vi "String To Number(I32).vi"(5 "String":string) -> (0 "Numeric(I32)":i32)   [LabVIEW 2017]
uses:
  581c0f11-9c78-43f6-8d57-08c5360404ff.vi
  4eae6f33-c0f2-4f9a-9685-dff6b581849e.vi
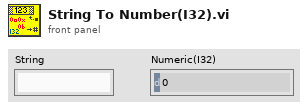
[diagram p1: front panel]
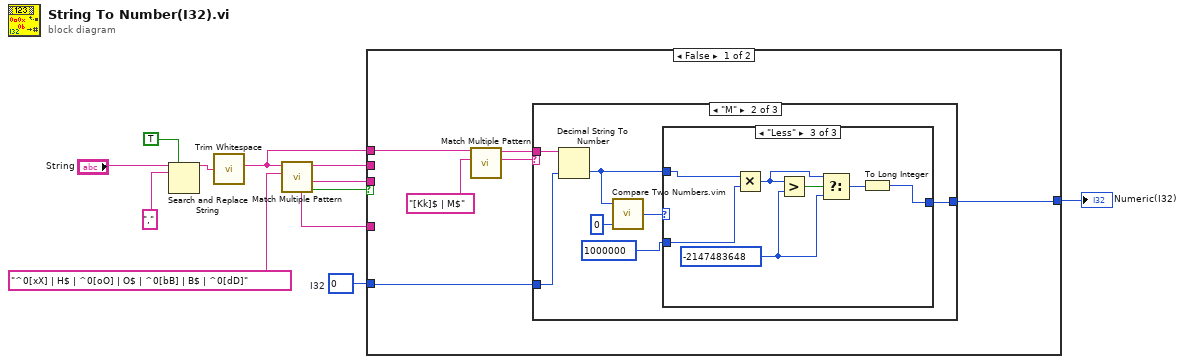
[diagram p0: block diagram]
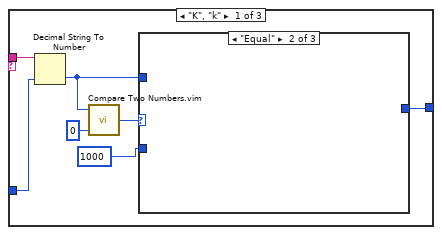
[diagram p2: hidden frame]
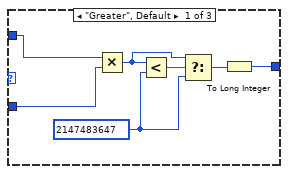
[diagram p3: hidden frame]
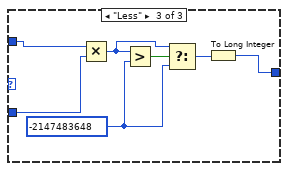
[diagram p4: hidden frame]
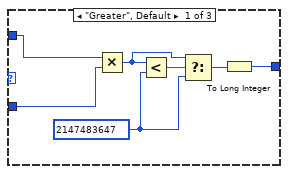
[diagram p5: hidden frame]
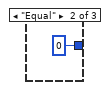
[diagram p6: hidden frame]
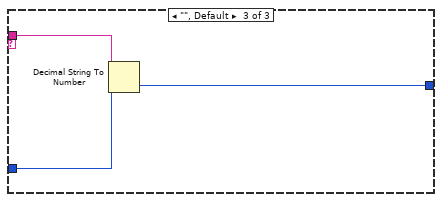
[diagram p7: hidden frame]
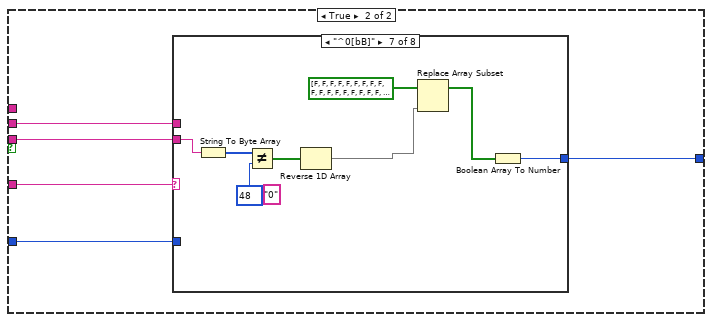
[diagram p8: hidden frame]
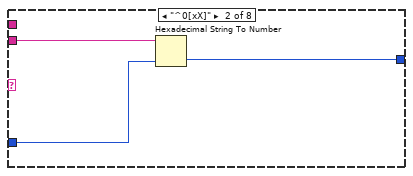
[diagram p10: hidden frame]
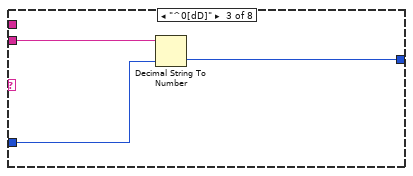
[diagram p11: hidden frame]
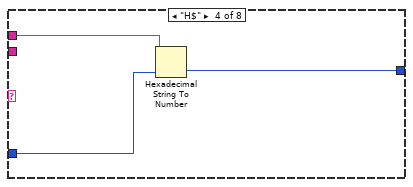
[diagram p12: hidden frame]
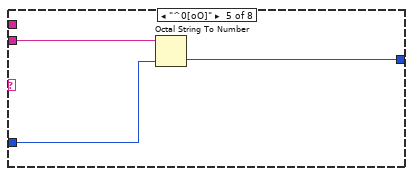
[diagram p13: hidden frame]
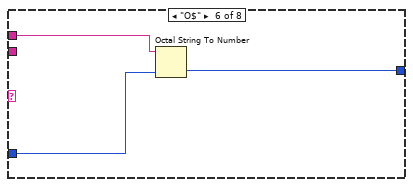
[diagram p14: hidden frame]
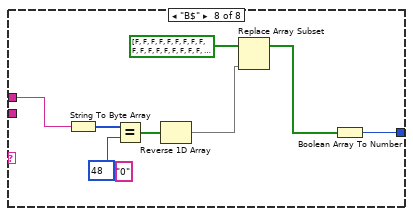
[diagram p15: hidden frame]
diagram:
  w1 = 0  # I32
  n1 = Search and Replace String(replace all?=TRUE ("replace all? (F)"), input string="String", search string=",") -> (result string=w9:string)  [unwired: 5 in, 3 out]
  n2 = call <vilib>:"Trim Whitespace.vi"("string"=w9) -> ("trimmed string"=w2:string)  [unwired: 1 in]
  n3 = call "Match Multiple Pattern.vi"("regular expression"="^0[xX] | H$ | ^0[oO] | O$ | ^0[bB] | B$ | ^0[dD]", "string"=w2) -> ("Found?"=w7:bool, "after substring"=w5:string, "before substring"=w4:string, "pattern matched"=w6:string)  [unwired: 5 in, 1 out]
  n4 = case shown="False" w7 {
    tunnel: w6 -> [_ w69]
    tunnel: w5 -> [_ w68]
    tunnel: w4 -> [_ w67]
    tunnel: [w13 w66] -> w3
    tunnel: w2 -> [w15 _]
    tunnel: w1 -> [w14 w65]
    frame False {
      n5 = call "Match Multiple Pattern.vi"("regular expression"="[Kk]$ | M$", "string"=w15) -> ("match substring"=w17:string, "before substring"=w16:string)  [unwired: 5 in, 3 out]
      n6 = case shown="\"M\"" w17 {
        tunnel: [w22 w43 w64] -> w13
        tunnel: w14 -> [w21 w42 w63]
        tunnel: w16 -> [w25 w46 w62]
        frame "K", "k" {
          n7 = Decimal String To Number(string=w25, default (0L)=w21) -> (number=w20:i32)  [unwired: 1 in, 1 out]
          n8 = call "Compare Two Numbers.vim"("Ref"=0, "Number"=w20) -> ("Result"=w23:enum16{"Greater", "Equal", "Less"})  [unwired: 1 in, 2 out]
          n9 = case shown="\"Equal\"" w23 {
            tunnel: [w26 _ w34] -> w22
            tunnel: w20 -> [w29 _ w35]
            tunnel: u64 1000 ("y") -> [w28 _ w33]
            frame "Greater", Default {
              w30 = 2147483647 ("y")
              n10 = Multiply(x=w29, y=w28) -> (x*y=w31:u64)
              n11 = Less?(x=w31, y=w30) -> (x < y?=w32:bool)
              n12 = Select(t=w31, s=w32, f=w30) -> (s? t:f=w27:u64)
              n13 = To Long Integer(number=w27) -> (32bit integer=w26:i32)
            }
            frame "Equal" {
            }
            frame "Less" {
              w37 = -2147483648 ("y")
              n14 = Multiply(x=w35, y=w33) -> (x*y=w38:u64)
              n15 = Greater?(x=w38, y=w37) -> (0:w39:bool)
              n16 = Select(t=w38, s=w39, f=w37) -> (s? t:f=w36:u64)
              n17 = To Long Integer(number=w36) -> (32bit integer=w34:i32)
            }
          }
        }
        frame "M" {
          n18 = Decimal String To Number(string=w46, default (0L)=w42) -> (number=w41:i32)  [unwired: 1 in, 1 out]
          n19 = call "Compare Two Numbers.vim"("Ref"=0, "Number"=w41) -> ("Result"=w44:enum16{"Greater", "Equal", "Less"})  [unwired: 1 in, 2 out]
          n20 = case shown="\"Less\"" w44 {
            tunnel: [w48 0 w56] -> w43
            tunnel: w41 -> [w50 _ w57]
            tunnel: i64 1000000 ("y") -> [w47 _ w55]
            frame "Greater", Default {
              w51 = 2147483647 ("y")
              n21 = Multiply(x=w50, y=w47) -> (x*y=w52:i64)
              n22 = Less?(x=w52, y=w51) -> (x < y?=w53:bool)
              n23 = Select(t=w52, s=w53, f=w51) -> (s? t:f=w49:i64)
              n24 = To Long Integer(number=w49) -> (32bit integer=w48:i32)
            }
            frame "Equal" {
            }
            frame "Less" {
              w59 = -2147483648 ("y")
              n25 = Multiply(x=w57, y=w55) -> (x*y=w60:i64)
              n26 = Greater?(x=w60, y=w59) -> (0:w61:bool)
              n27 = Select(t=w60, s=w61, f=w59) -> (s? t:f=w58:i64)
              n28 = To Long Integer(number=w58) -> (32bit integer=w56:i32)
            }
          }
        }
        frame "", Default {
          n29 = Decimal String To Number(string=w62, default (0L)=w63) -> (number=w64:i32)  [unwired: 1 in, 1 out]
        }
      }
    }
    frame True {
      n30 = case shown="\"^0[bB]\"" w69 {
        tunnel: w68 -> [_ w73 w76 _ w82 _ w92 _]
        tunnel: w67 -> [_ _ _ w78 _ w84 _ w98]
        tunnel: [w70 w72 w75 w79 w81 w85 w93 w101] -> w66
        tunnel: w65 -> [w70 w71 w74 w77 w80 w83 _ _]
        frame Default {
        }
        frame "^0[xX]" {
          n31 = Hexadecimal String To Number(string=w73, default (0uL)=w71) -> (number=w72:i32)  [unwired: 1 in, 1 out]
        }
        frame "^0[dD]" {
          n32 = Decimal String To Number(string=w76, default (0L)=w74) -> (number=w75:i32)  [unwired: 1 in, 1 out]
        }
        frame "H$" {
          n33 = Hexadecimal String To Number(string=w78, default (0uL)=w77) -> (number=w79:i32)  [unwired: 1 in, 1 out]
        }
        frame "^0[oO]" {
          n34 = Octal String To Number(2:w80, 4:w82) -> (0:w81:i32)  [unwired: 1 in, 1 out]
        }
        frame "O$" {
          n35 = Octal String To Number(2:w83, 4:w84) -> (0:w85:i32)  [unwired: 1 in, 1 out]
        }
        frame "^0[bB]" {
          (unwired) "0" ("search string")
          n36 = String To Byte Array(string=w92) -> (unsigned byte array=w91:u8[])
          n37 = Not Equal?(x=w91, y=u8 48) -> (x != y?=w89:bool[])
          n38 = Reverse 1D Array(array=w89) -> (reversed array=w87:bool[])
          n39 = Replace Array Subset(array=bool[] [FALSE, FALSE, FALSE, FALSE, FALSE, FALSE, FALSE, FALSE, FALSE, FALSE, FALSE, FALSE, FALSE, FALSE, FALSE, FALSE, FALSE, FALSE, FALSE, FALSE, FALSE, FALSE, FALSE, FALSE, FALSE, FALSE, FALSE, FALSE, FALSE, FALSE, FALSE, FALSE], new element=w87) -> (w86:bool[])  [unwired: 1 in]
          n40 = Boolean Array To Number(Boolean array=w86) -> (number=w93:i32)
        }
        frame "B$" {
          (unwired) "0" ("search string")
          n41 = String To Byte Array(string=w98) -> (unsigned byte array=w100:u8[])
          n42 = Equal?(x=w100, y=u8 48) -> (x = y?=w99:bool[])
          n43 = Reverse 1D Array(array=w99) -> (reversed array=w95:bool[])
          n44 = Replace Array Subset(array=bool[] [FALSE, FALSE, FALSE, FALSE, FALSE, FALSE, FALSE, FALSE, FALSE, FALSE, FALSE, FALSE, FALSE, FALSE, FALSE, FALSE, FALSE, FALSE, FALSE, FALSE, FALSE, FALSE, FALSE, FALSE, FALSE, FALSE, FALSE, FALSE, FALSE, FALSE, FALSE, FALSE], new element=w95) -> (w94:bool[])  [unwired: 1 in]
          n45 = Boolean Array To Number(Boolean array=w94) -> (number=w101:i32)
        }
      }
    }
  }
  "Numeric(I32)" <- w3
